vi "字符串整理-文件名.vi"(6 "删除字符串数组":string[](array[string])=["\\", "/", ":", "*", "?", "\"", "<", ">", "|"], 10 "输入字符串":string) -> (2 "结果字符串":string)   [LabVIEW 2025]
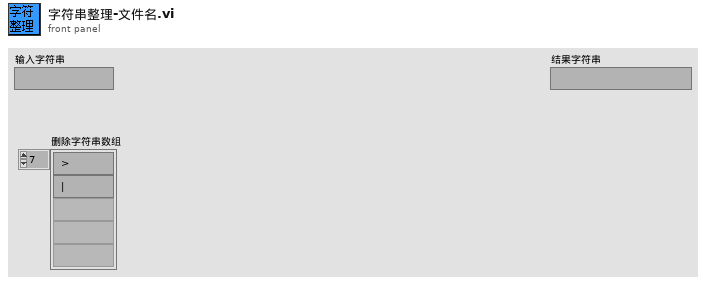
[diagram p1: front panel]
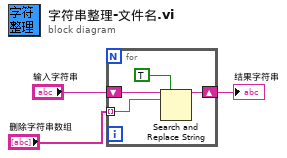
[diagram p0: block diagram]
diagram:
  n1 = for {
    tunnel: "删除字符串数组" -> [w5] mode=indexing
    shift-right: [w4] -> w1
    shift-left: "输入字符串" -> [w6]
    n2 = Search and Replace String(replace all?=TRUE ("替换全部？(F)"), input string=w6, search string=w5) -> (result string=w4:string)  [unwired: 5 in, 3 out]
  }
  "结果字符串" <- w1
